vi "calibracion.vi"(0 "voltaje PH 1":dbl, 1 "voltaje PH 2":dbl, 2 "Voltaje OD 1":dbl, 3 "Voltaje OD 2":dbl, 6 "aPh1":dbl=0.5407 format="%#_13g", 7 "aOD1":dbl=0.5407 format="%#_13g", 8 "bPh1":dbl=1.2462 format="%#_13g", 9 "bOD1":dbl=1.2462 format="%#_13g", 10 "aPh2":dbl=0.5407 format="%#_13g", 11 "aOD2":dbl=0.5407 format="%#_13g", 12 "bPh2":dbl=1.2462 format="%#_13g", 13 "bOD2":dbl=1.2462 format="%#_13g") -> (14 "PH 1":dbl, 15 "PH 2":dbl, 16 "OD 1":dbl, 17 "OD 2":dbl)   [LabVIEW 2013]
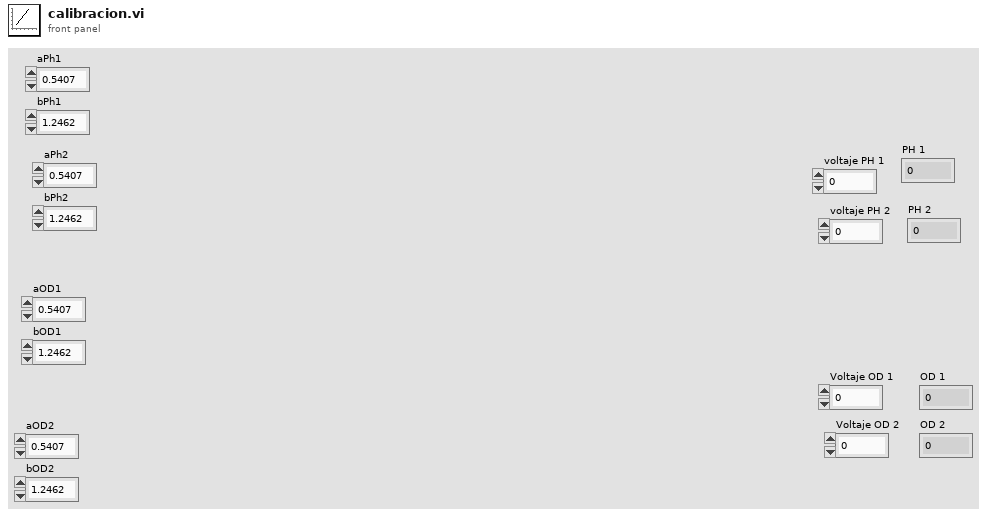
[diagram p1: front panel]
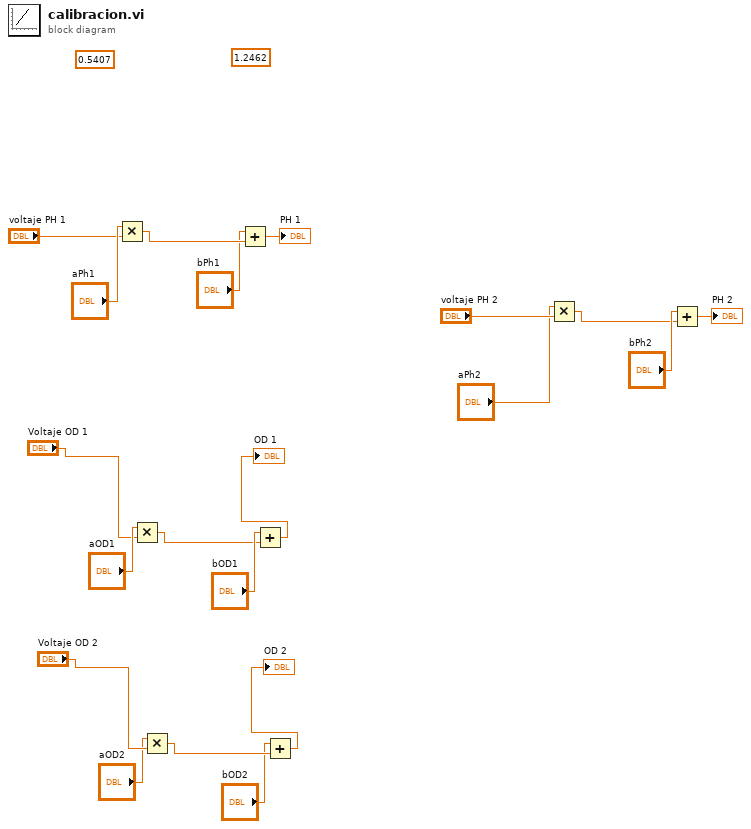
[diagram p0: block diagram]
diagram:
  (unwired) 0.5407 ("x")
  (unwired) 1.2462 ("y")
  n1 = Multiply(x="aPh1", y="voltaje PH 1") -> (x*y=w17:dbl)
  n2 = Multiply(x="aOD1", y="Voltaje OD 1") -> (x*y=w14:dbl)
  n3 = Multiply(x="aOD2", y="Voltaje OD 2") -> (x*y=w7:dbl)
  n4 = Add(x="bPh1", y=w17) -> (x+y=→"PH 1":dbl)
  n5 = Add(x="bOD1", y=w14) -> (x+y=→"OD 1":dbl)
  n6 = Add(x="bOD2", y=w7) -> (x+y=→"OD 2":dbl)
  n7 = Multiply(x="aPh2", y="voltaje PH 2") -> (x*y=w4:dbl)
  n8 = Add(x="bPh2", y=w4) -> (x+y=→"PH 2":dbl)
